vi "G4SubTemplate_Simple_4x4x4_WriteAttribute.vi"(0 "reference in":refnum<class "G4SubTemplate_Simple_4x4x4.lvclass">, 5 "Error In":errorcluster) -> (14 "reference out":refnum<class "G4SubTemplate_Simple_4x4x4.lvclass">, 19 "Error Out":errorcluster)   [LabVIEW 2020]
uses:
  G4SubTemplate_Simple_4x4x4.lvclass
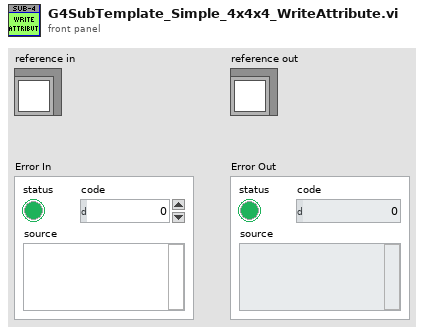
[diagram p1: front panel]
types:
  T1 = typedef "G4SubTemplate_Simple_4x4x4.lvclass/ObjectAttributes.ctl" = cluster{"Attribute1":dbl}
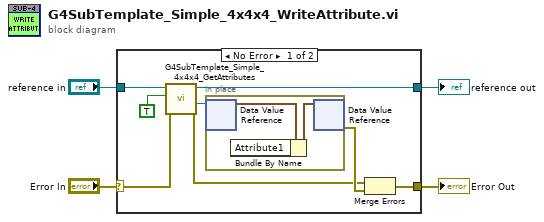
[diagram p0: block diagram]
diagram:
  n1 = case shown="No Error" "Error In" {
    selector: "Error In" -> [w10 w16]
    tunnel: [w5 w16] -> w3
    tunnel: [w11 w15] -> w1
    tunnel: "reference in" -> [w12 w15]
    frame No Error {
      n2 = call "G4SubTemplate_Simple_4x4x4_GetAttributes.vi"("Error In"=w10, "OnlyGetDvrReference(False)"=TRUE, "reference in"=w12) -> ("Error Out"=w6:errorcluster, "DataRef"=w7:refnum<data-value>, "reference out"=w11:refnum<class "G4SubTemplate_Simple_4x4x4.lvclass">)  [unwired: 5 in, 1 out]
      n3 = in-place {
        n4 = in-place-dvr #1(w7) -> (w13:T1)  [unwired: 1 out]
        n5 = Bundle By Name(cluster=w13) -> (w14:T1)  [unwired: 1 in]
        n6 = in-place-dvr #1(w14) -> (w8:errorcluster)  [unwired: 1 out]
      }
      n7 = Merge Errors(w6, w8) -> (w5:errorcluster)
    }
    frame Error {
    }
  }
  "Error Out" <- w3
  "reference out" <- w1
